vi "Get Device Settings from INI File.vi"(8 "error in (no error)":errorcluster) -> (0 "error out":errorcluster, 3 "Device Settings":T1[](array[typedef]))   [LabVIEW 2021]
uses:
  TypeDefs/Device Settings.ctl
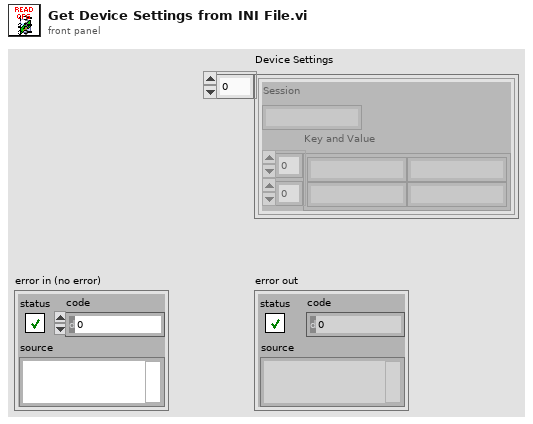
[diagram p1: front panel]
types:
  T1 = typedef "Device Settings.ctl" = cluster{"Session":string, "Key and Value":string[][]}
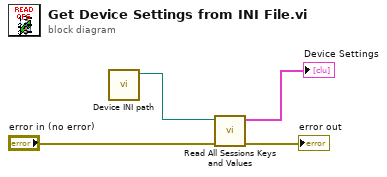
[diagram p0: block diagram]
diagram:
  n1 = call "Device INI path.vi"() -> ("appended path"=w2:path)  [unwired: 11 in]
  n2 = call "Read All Sessions Keys and Values.vi"("error in (no error)"="error in (no error)", "appended path"=w2) -> ("error out"=→"error out":errorcluster, "Device Settings"=→"Device Settings":T1[])  [unwired: 8 in]
